vi "upload.file.vi"(8 "error in":errorcluster, 10 "File":path, 11 "Nominal Client in":refnum<class "Nominal Client.lvclass">) -> (0 "error out":errorcluster, 2 "Path to S3 File":string, 3 "Nominal Client out":refnum<class "Nominal Client.lvclass">)   [LabVIEW 2020, in "Nominal Client.lvclass"]
doc: "Uploads a file to S3. Intended for smaller files."
uses:
  Nominal Client.lvclass
  Nominal Client.lvclass/Nominal Client.ctl
  nominal types/workspace/workspace.lvclass
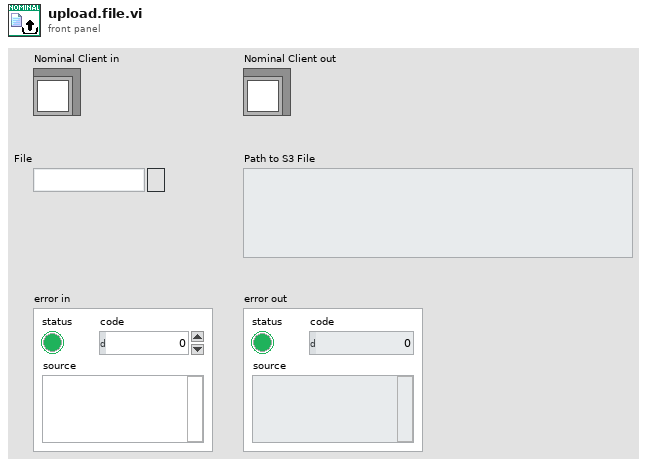
[diagram p1: front panel]
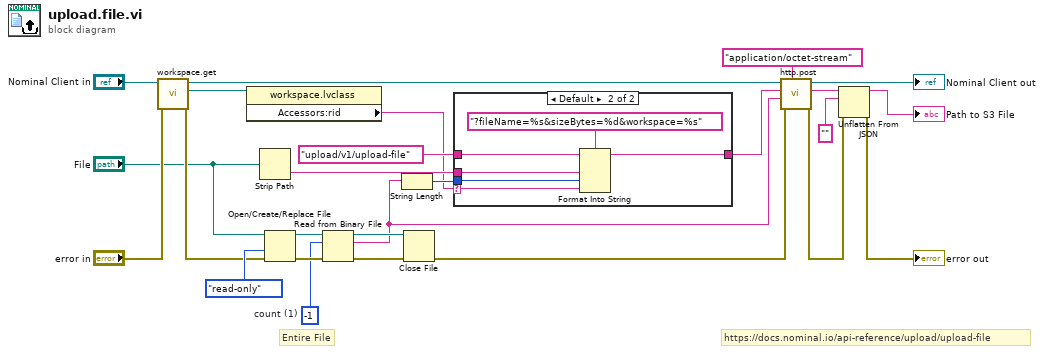
[diagram p0: block diagram]
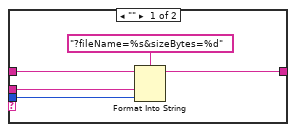
[diagram p2: hidden frame]
diagram:
  w20 = -1  # count (1)
  # "https://docs.nominal.io/api-reference/upload/upload-file"
  # "Entire File"
  n1 = call "workspace.get.vi"("error in"="error in", "Nominal Client in"="Nominal Client in") -> ("error out"=w4:errorcluster, "workspace"=w2:refnum<class "workspace.lvclass">, "Nominal Client out"=w7:refnum<class "Nominal Client.lvclass">)  [unwired: 7 in]
  n2 = property class="workspace.lvclass"(reference=w2) -> ("Accessors:rid"=w1:string)  [unwired: 1 in, 2 out]
  n3 = Strip Path(path="File") -> (name=w9:string)  [unwired: 1 out]
  n4 = Open/Create/Replace File(file path (use dialog)="File", error in=w4, access (0:read/write)=enum16{"read/write", "read-only", "write-only"}."read-only") -> (refnum out=w25:refnum<file>, error out=w24:errorcluster)  [unwired: 3 in, 1 out]
  n5 = Read from Binary File(8:w24, 10:w20, 11:w25) -> (0:w22:errorcluster, 2:w16:string, 3:w23:refnum<file>)  [unwired: 3 in, 1 out]
  n6 = String Length(string=w16) -> (length=w18:i32)
  n7 = Close File(refnum=w23, error in=w22) -> (error out=w19:errorcluster)  [unwired: 1 out]
  n8 = case shown="Default" w1 {
    selector: w1 -> [_ w32]
    tunnel: w18 -> [w30 w36]
    tunnel: "upload/v1/upload-file" ("Path") -> [w29 w35]
    tunnel: w9 -> [w28 w34]
    tunnel: [w27 w33] -> w6
    frame "" {
      n9 = Format Into String(format string="?fileName=%s&sizeBytes=%d" ("Path"), initial string=w29, w28, w30) -> (resulting string=w27:string)  [unwired: 1 in, 1 out]
    }
    frame Default {
      n10 = Format Into String(format string="?fileName=%s&sizeBytes=%d&workspace=%s" ("Path"), initial string=w35, w34, w36, w32) -> (resulting string=w33:string)  [unwired: 1 in, 1 out]
    }
  }
  n11 = call "http.post.vi"("Content Type"="application/octet-stream", "error in"=w19, "Request body"=w16, "Path"=w6, "Nominal Client in"=w7) -> ("error out"=w11:errorcluster, "Response"=w14:string, "Nominal Client out"=→"Nominal Client out":refnum<class "Nominal Client.lvclass">)  [unwired: 3 in, 1 out]
  n12 = Unflatten From JSON(JSON string=w14, type and defaults="", error in (no error)=w11) -> (value=→"Path to S3 File":string, error out=→"error out":errorcluster)  [unwired: 4 in]
